vi "KYFG Camera Close.vi"(8 "error in (no error)":errorcluster, 11 "camHandle":u32) -> (0 "error out":errorcluster)   [LabVIEW 2023, in "KYFGLib_lv.lvlib"]
doc: "KYFG_API FGSTATUS KYFG_CameraClose(CAMHANDLE camHandle);"
uses:
  KYFGLib_lv.lvlib
  KYFGLib.dll
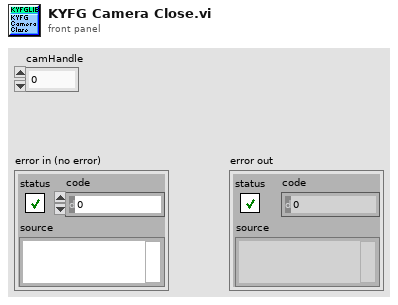
[diagram p1: front panel]
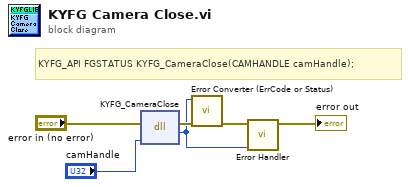
[diagram p0: block diagram]
diagram:
  # "KYFG_API FGSTATUS KYFG_CameraClose(CAMHANDLE camHandle);"
  n1 = dll-call lib="KYFGLib.dll" fn="KYFG_CameraClose"(error in="error in (no error)", "camHandle"="camHandle") -> (error out=w4:errorcluster, "return type"=w3:u32)  [unwired: 3 in, 1 out]
  n2 = call "Error Converter (ErrCode or Status).vi"("error in (no error)"=w4, "error code"=w3) -> ("error out"=w2:errorcluster)  [unwired: 9 in]
  n3 = call "Error Handler.vi"("Return Code"=w3, "Error In"=w2) -> ("Error Out"=→"error out":errorcluster)  [unwired: 9 in]
